vi "Calculate.vi"(7 "Conversion":refnum<k21>, 8 "error in (no error)":errorcluster, 9 "PCL dt":dbl, 10 "Values":dbl[](array[numeric]), 11 "Frame Configuration":T1 {"CRC"."Data Type" items=["Signed", "Unsigned", "IEEE Float"]; "Rolling Counter"."Data Type" items=["Signed", "Unsigned", "IEEE Float"]; "Input Channels"."Data Type" items=["Signed", "Unsigned", "IEEE Float"]}) -> (0 "error out":errorcluster, 1 "ProtectionValue":dbl, 2 "Rolling Counter":dbl, 3 "Frame Configuration":T1 {"CRC"."Data Type" items=["Signed", "Unsigned", "IEEE Float"]; "Rolling Counter"."Data Type" items=["Signed", "Unsigned", "IEEE Float"]; "Input Channels"."Data Type" items=["Signed", "Unsigned", "IEEE Float"]})   [LabVIEW 2015, in "Protection and Rolling Counter Addon Engine.lvlib"]
uses:
  Protection and Rolling Counter Addon Engine.lvlib
  Shared/Types/FrameConfiguration.ctl
  Shared/Types/InputChannelConfiguration.ctl
  Shared/Types/Protection Type.ctl
  <vilib>/xnet/xnet.llb/XNET Convert (Signal to Frame Raw).vi
  Shared/Protection and Rolling Counter Addon Shared.lvlib
panel:
  out "PCLIterations":dbl
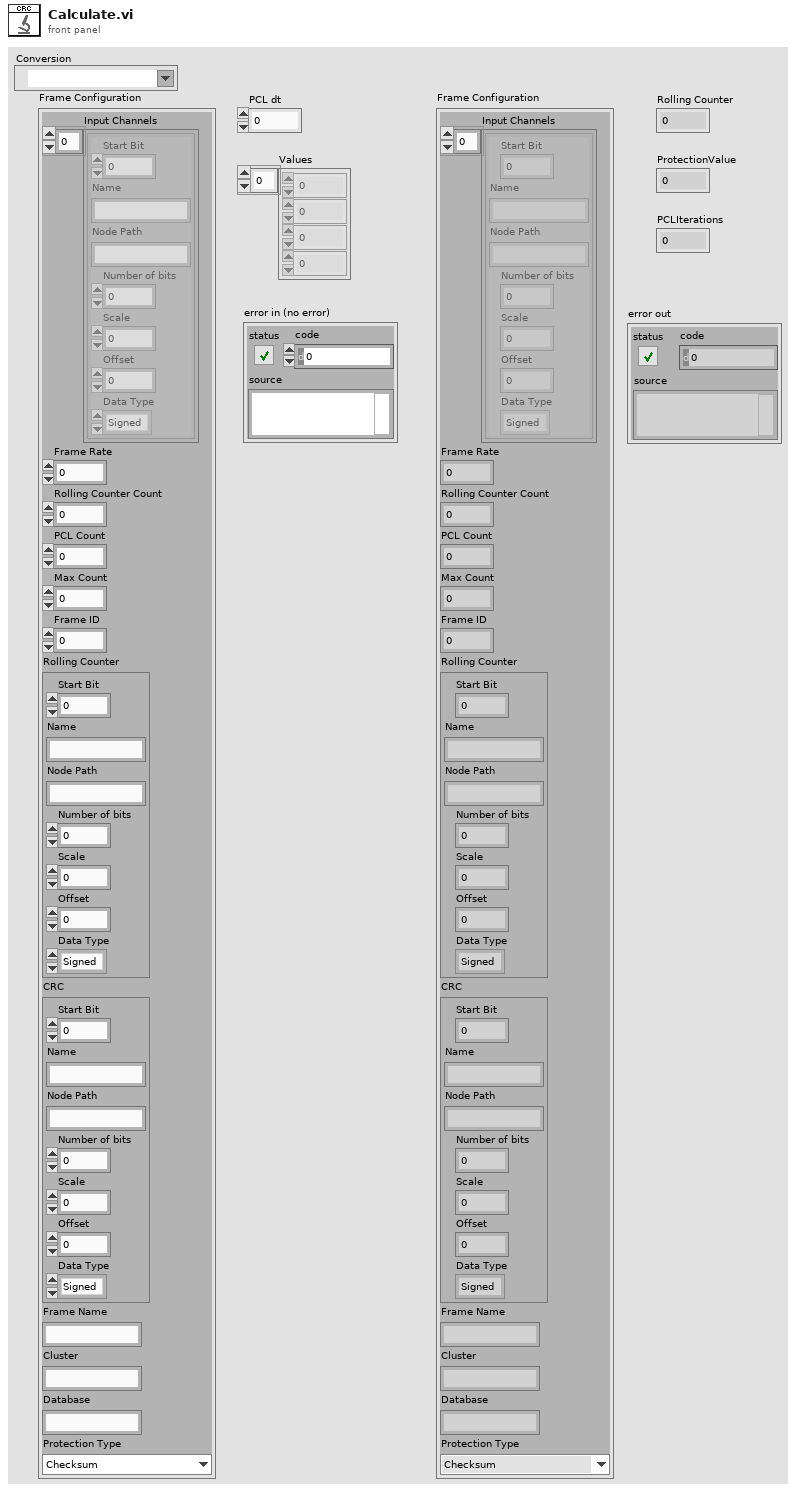
[diagram p1: front panel]
types:
  T1 = typedef "Protection and Rolling Counter Addon Shared.lvlib/FrameConfiguration.ctl" = cluster{"Input Channels":T2[], "Frame Rate":dbl, "Rolling Counter Count":dbl, "PCL Count":u64, "Max Count":dbl, "Frame ID":u32, "Rolling Counter":T2, "CRC":T2, "Frame Name":string, "Cluster":string, "Database":string, "Protection Type":T3}
  T2 = typedef "Protection and Rolling Counter Addon Shared.lvlib/InputChannelConfiguration.ctl" = cluster{"Start Bit":i32, "Name":string, "Node Path":string, "Number of bits":i32, "Scale":dbl, "Offset":dbl, "Data Type":u32}
  T3 = typedef "Protection and Rolling Counter Addon Shared.lvlib/Protection Type.ctl" = enum16{"Checksum", "CRC", "None (Counter Only)"}
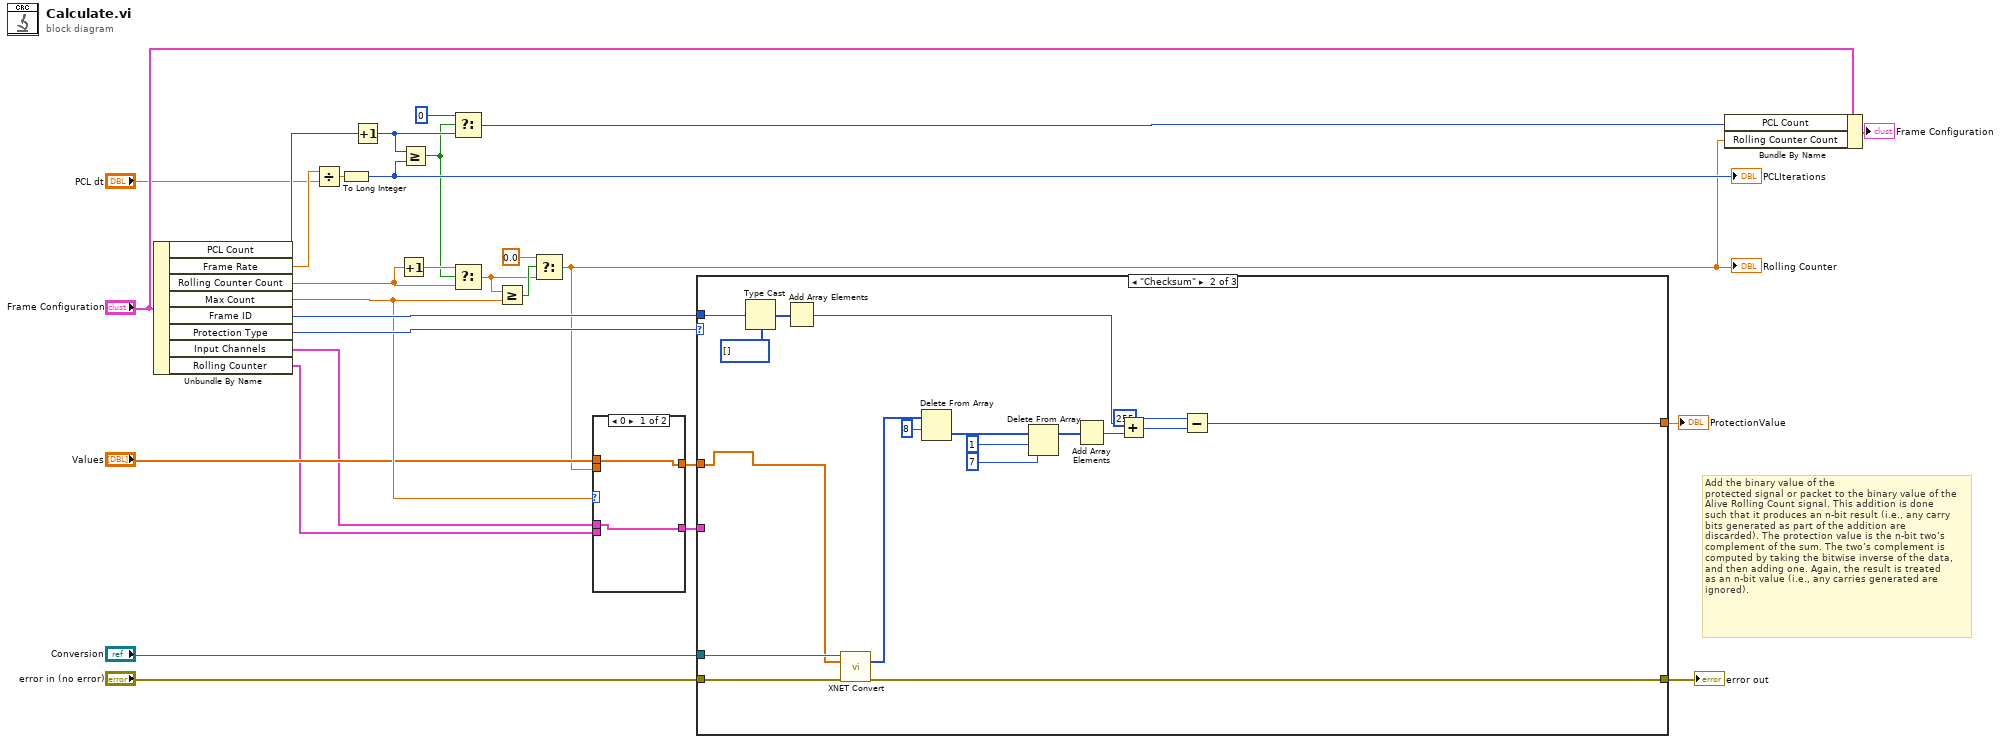
[diagram p0: block diagram]
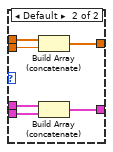
[diagram p2: hidden frame]
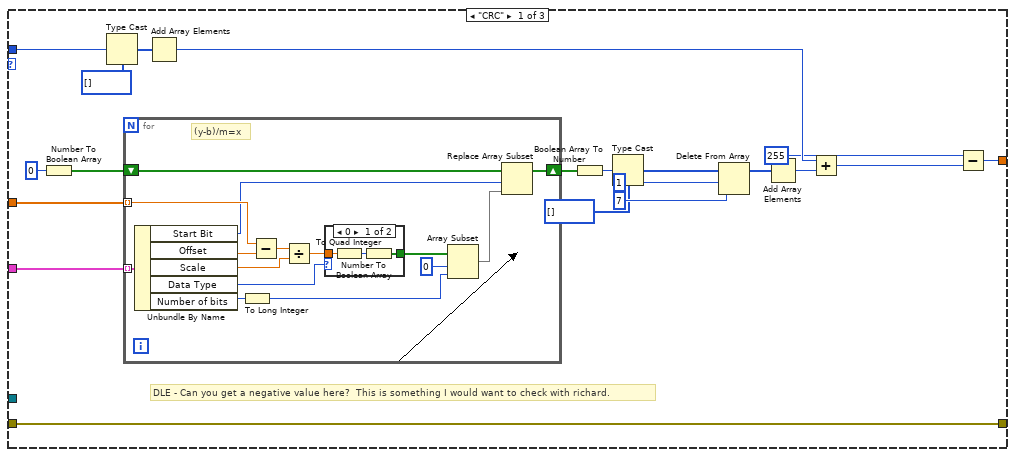
[diagram p3: hidden frame]
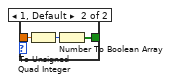
[diagram p4: hidden frame]
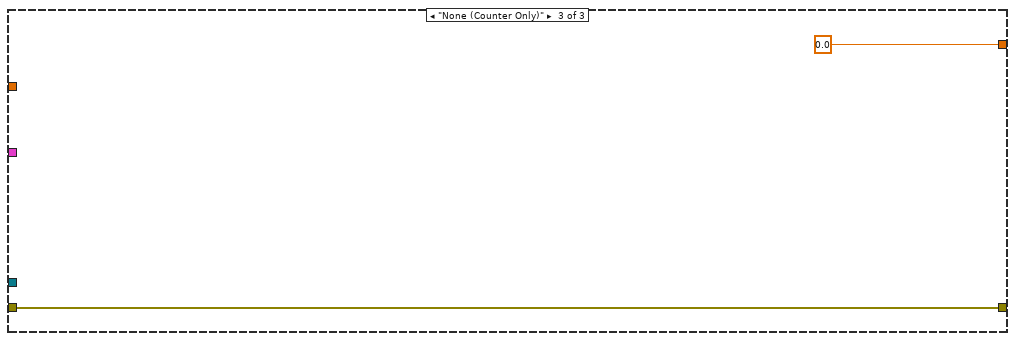
[diagram p5: hidden frame]
diagram:
  # "Add the binary value of the\nprotected signal or packet to the binary value of the\nAlive Rolling Count signal. This addition is done\nsuch that it produces an n-bit result (i.e., any carry\nbits generated as part of the addition are\ndiscarded). The protection value is the n-bit two’s\ncomplement of the sum. The two’s complement is\ncomputed by taking the bitwise inverse of the data,\nand then adding one. Again, the result is treated\nas an n-bit value (i.e., any carries generated are\nignored)."
  n1 = Unbundle By Name("Frame Configuration") -> ("PCL Count"=w24:u64, "Frame Rate"=w21:dbl, "Rolling Counter Count"=w22:dbl, "Max Count"=w7:dbl, "Frame ID"=w13:u32, "Protection Type"=w8:T3, "Input Channels"=w4:T2[], "Rolling Counter"=w3:T2)
  n2 = Divide(x=w21, y="PCL dt") -> (x/y=w29:dbl)
  n3 = To Long Integer(number=w29) -> (32bit integer=w18:i32)
  "PCLIterations" <- w18
  n4 = Increment(x=w24) -> (x+1=w17:u64)
  n5 = Increment(x=w22) -> (x+1=w28:dbl)
  n6 = Greater Or Equal?(x=w17, y=w18) -> (x >= y?=w14:bool)
  n7 = Select(t=u64 0, s=w14, f=w17) -> (s? t:f=w15:u64)
  n8 = Select(t=w28, s=w14, f=w22) -> (s? t:f=w26:dbl)
  n9 = Greater Or Equal?(x=w26, y=w7) -> (x >= y?=w27:bool)
  n10 = Select(t=0.0, s=w27, f=w26) -> (s? t:f=w5:dbl)
  "Rolling Counter" <- w5
  n11 = case shown="0" w7 {
    tunnel: "Values" -> [w30 w37]
    tunnel: w5 -> [_ w36]
    tunnel: w4 -> [w31 w35]
    tunnel: w3 -> [_ w34]
    tunnel: [w31 w33] -> w2
    tunnel: [w30 w32] -> w1
    frame 0 {
    }
    frame Default {
      n12 = Build Array (concatenate)(w37, w36) -> (w32:dbl[])
      n13 = Build Array (concatenate)(w35, w34) -> (w33:T2[])
    }
  }
  n14 = case shown="\"Checksum\"" w8 {
    tunnel: w13 -> [w51 w90 _]
    tunnel: [w46 w85 0.0] -> w12
    tunnel: "error in (no error)" -> [w40 w84 w98]
    tunnel: [w40 w83 w98] -> w10
    tunnel: "Conversion" -> [_ w82 _]
    tunnel: w2 -> [w38 _ _]
    tunnel: w1 -> [w39 w79 _]
    frame "CRC" {
      # "DLE - Can you get a negative value here?  This is something I would want to check with richard."
      n15 = Number To Boolean Array(number=u64 0) -> (Boolean array=w45:bool[])
      n16 = Type Cast(type=u8[] [], x=w51) -> (*(type *) &x=w50:u8[])
      n17 = for {
        tunnel: w38 -> [w72] mode=indexing
        shift-right: [w63] -> w43
        shift-left: w45 -> [w65]
        tunnel: w39 -> [w62] mode=indexing
        # "(y-b)/m=x"
        n18 = Unbundle By Name(w72) -> ("Start Bit"=w59:i32, "Offset"=w71:dbl, "Scale"=w69:dbl, "Data Type"=w61:u32, "Number of bits"=w67:i32)
        n19 = To Long Integer(number=w67) -> (32bit integer=w58:i32)
        n20 = Subtract(x=w62, y=w71) -> (x-y=w70:dbl)
        n21 = Divide(x=w70, y=w69) -> (x/y=w68:dbl)
        n22 = case shown="0" w61 {
          tunnel: w68 -> [w75 w78]
          tunnel: [w73 w76] -> w60
          frame 0 {
            n23 = To Quad Integer(1:w75) -> (0:w74:i64)
            n24 = Number To Boolean Array(number=w74) -> (Boolean array=w73:bool[])
          }
          frame 1, Default {
            n25 = To Unsigned Quad Integer(1:w78) -> (0:w77:u64)
            n26 = Number To Boolean Array(number=w77) -> (Boolean array=w76:bool[])
          }
        }
        n27 = Array Subset(array=w60, index=0, length=w58) -> (w64:bool[])
        n28 = Replace Array Subset(array=w65, new element=w64, index=w59) -> (w63:bool[])
      }
      n29 = Add Array Elements(numeric array=w50) -> (sum=w49:u8)
      n30 = Boolean Array To Number(Boolean array=w43) -> (number=w42:u64)
      n31 = Type Cast(type=u8[] [], x=w42) -> (*(type *) &x=w57:u8[])
      n32 = Delete From Array(array=w57, length=1, index=7) -> (array with subset deleted=w54:u8[])  [unwired: 1 out]
      n33 = Add Array Elements(numeric array=w54) -> (sum=w53:u8)
      n34 = Add(x=w49, y=w53) -> (x+y=w48:u8)
      n35 = Subtract(x=u8 255, y=w48) -> (x-y=w46:u8)
    }
    frame "Checksum" {
      n36 = Type Cast(type=u8[] [], x=w90) -> (*(type *) &x=w89:u8[])
      n37 = Add Array Elements(numeric array=w89) -> (sum=w88:u8)
      n38 = call-poly <vilib>:"XNET Convert.vi"("session in"=w82, "signal data"=w79, "error in (no error)"=w84) -> ("frame data"=w80:u8[], "error out"=w83:errorcluster)  [unwired: 10 in, 1 out]
      n39 = Delete From Array(array=w80, length=8) -> (deleted portion=w96:u8[])  [unwired: 1 in, 1 out]
      n40 = Delete From Array(array=w96, length=1, index=7) -> (array with subset deleted=w93:u8[])  [unwired: 1 out]
      n41 = Add Array Elements(numeric array=w93) -> (sum=w92:u8)
      n42 = Add(x=w88, y=w92) -> (x+y=w87:u8)
      n43 = Subtract(x=u8 255, y=w87) -> (x-y=w85:u8)
    }
    frame "None (Counter Only)" {
    }
  }
  "ProtectionValue" <- w12
  "error out" <- w10
  n44 = Bundle By Name(cluster="Frame Configuration", "PCL Count"=w15, "Rolling Counter Count"=w5) -> (→"Frame Configuration":T1)
